vi "PicoScope2000aOpen.vi"(4 "Serial Number":string, 6 "Use Serial Number":bool, 7 "error in (no error)":errorcluster) -> (0 "Max Adc value":i16, 1 "handle":i16, 3 "error out":errorcluster, 5 "Device Info":T1)   [LabVIEW 2010]
doc: "This VI opens a PicoScope 3000a/b and returns a handle to the device."
uses:
  ps2000a.dll
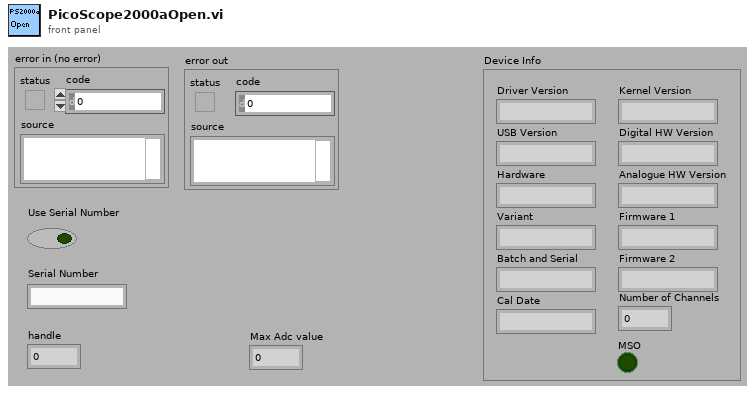
[diagram p1: front panel]
types:
  T1 = cluster{"Driver Version":string, "USB Version":string, "Hardware":string, "Variant":string, "Batch and Serial":string, "Cal Date":string, "Kernel Version":string, "Digital HW Version":string, "Analogue HW Version":string, "Firmware 1":string, "Firmware 2":string, "MSO":bool, "Number of Channels":i16}
  T2 = cluster{"Driver Version":string, "USB Version":string, "Hardware":string, "Variant":string, "Batch and Serial":string, "Cal Date":string, "Kernel Version":string, "Digital HW Version":string, "Analogue HW Version":string, "Firmware 1":string, "Firmware 2":string}
  T3 = cluster{"Driver Version":string, "USB Version":string, "Hardware":string, "Variant":string, "Batch and Serial":string, "Cal Date":string, "Kernel Version":string, "Digital HW Version":string, "Analogue HW Version":string, "Firmware 1":string, "Firmware 2":string, bool, i16}
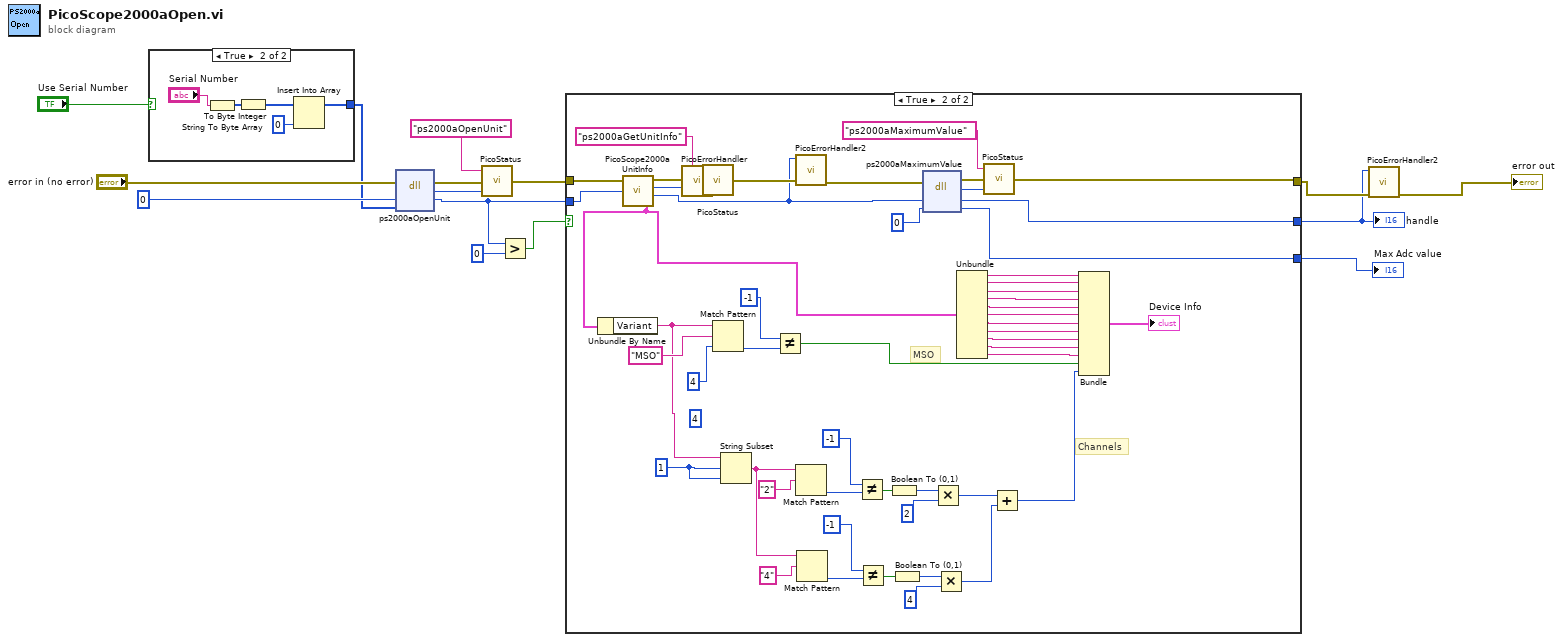
[diagram p0: block diagram]
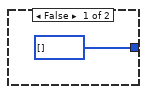
[diagram p2: hidden frame]
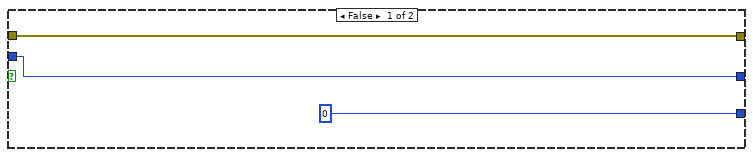
[diagram p3: hidden frame]
diagram:
  n1 = case shown="True" "Use Serial Number" {
    tunnel: [i8[] [] ("serial") w18] -> w1
    frame False {
    }
    frame True {
      n2 = String To Byte Array(string="Serial Number") -> (unsigned byte array=w21:u8[])
      n3 = To Byte Integer(number=w21) -> (8bit integer=w20:i8[])
      n4 = Insert Into Array(array=w20, new element=i8 0 ("new element/subarray")) -> (w18:i8[])  [unwired: 1 in]
    }
  }
  n5 = dll-call lib="ps2000a.dll" fn="ps2000aOpenUnit" ("ps3000.dll:_ps3000_open_unit@0")(error in="error in (no error)", "handle"=i16 0, "serial"=w1) -> (error out=w6:errorcluster, "PICO_STATUS"=w3:u32, "handle"=w2:i16)  [unwired: 3 in, 1 out]
  n6 = call "PicoStatus.vi"("PICO STATUS"=w3, "error in"=w6, "source"="ps2000aOpenUnit") -> ("error out"=w12:errorcluster)
  n7 = Greater?(x=w2, y=i16 0) -> (0:w14:bool)
  n8 = case shown="True" w14 {
    tunnel: w2 -> [w23 w73]
    tunnel: w12 -> [w24 w74]
    tunnel: [w24 w28] -> w10
    tunnel: [w23 w69] -> w8
    tunnel: [i16 0 ("value") w70] -> w11
    frame False {
    }
    frame True {
      w47 = 1 ("offset (0)")
      (unwired) 4 ("offset (0)")
      # "MSO"
      # "Channels"
      n9 = call "PicoScope2000aUnitInfo.vi"("error in (no error)"=w74, "handle in"=w73) -> ("error out"=w72:errorcluster, "PICO_STATUS"=w71:u32, "handle out"=w25:i16, "Unit Info"=w59:T2)  [unwired: 1 in]
      n10 = Unbundle By Name(w59) -> ("Variant"=w31:string)
      n11 = call "PicoStatus.vi"("PICO STATUS"=w71, "error in"=w72, "source"="ps2000aGetUnitInfo") -> ("error out"=w27:errorcluster)
      n12 = Match Pattern(string=w31, regular expression="MSO", offset (0)=4) -> (offset past match=w63:i32)  [unwired: 3 out]
      n13 = String Subset(string=w31, offset (0)=w47, length (rest)=w47) -> (substring=w40:string)
      n14 = Not Equal?(x=-1, y=w63) -> (x != y?=w60:bool)
      n15 = call "PicoErrorHandler2.vi"("error in (no error)"=w27, "handle In"=w25) -> ("error out"=w26:errorcluster)  [unwired: 9 in]
      n16 = Match Pattern(string=w40, regular expression="2") -> (offset past match=w45:i32)  [unwired: 1 in, 3 out]
      n17 = Match Pattern(string=w40, regular expression="4") -> (offset past match=w42:i32)  [unwired: 1 in, 3 out]
      n18 = Not Equal?(x=-1, y=w45) -> (x != y?=w37:bool)
      n19 = Not Equal?(x=-1, y=w42) -> (x != y?=w33:bool)
      n20 = Boolean To (0,1)(Boolean=w37) -> (0, 1=w36:i16)
      n21 = Boolean To (0,1)(Boolean=w33) -> (0, 1=w34:i16)
      n22 = dll-call lib="ps2000a.dll" fn="ps2000aMaximumValue"(error in=w26, "handle"=w25, "value"=i16 0) -> (error out=w67:errorcluster, "PICO_STATUS"=w66:u32, "handle"=w69:i16, "value"=w70:i16)  [unwired: 2 in, 1 out]
      n23 = Multiply(x=w36, y=i16 2) -> (x*y=w39:i16)
      n24 = Multiply(x=w34, y=i16 4) -> (x*y=w32:i16)
      n25 = Unbundle(w59) -> ("Driver Version"=w48:string, "USB Version"=w49:string, "Hardware"=w50:string, "Variant"=w51:string, "Batch and Serial"=w52:string, "Cal Date"=w53:string, "Kernel Version"=w54:string, "Digital HW Version"=w55:string, "Analogue HW Version"=w56:string, "Firmware 1"=w57:string, "Firmware 2"=w58:string)
      n26 = call "PicoStatus.vi"("PICO STATUS"=w66, "error in"=w67, "source"="ps2000aMaximumValue") -> ("error out"=w28:errorcluster)
      n27 = Add(x=w39, y=w32) -> (x+y=w30:i16)
      n28 = Bundle("Driver Version"=w48, "USB Version"=w49, "Hardware"=w50, "Variant"=w51, "Batch and Serial"=w52, "Cal Date"=w53, "Kernel Version"=w54, "Digital HW Version"=w55, "Analogue HW Version"=w56, "Firmware 1"=w57, "Firmware 2"=w58, w60, w30) -> (→"Device Info":T3)  [unwired: 1 in]
    }
  }
  "handle" <- w8
  "Max Adc value" <- w11
  n29 = call "PicoErrorHandler.vi"() -> ()  [unwired: 1 in, 1 out]
  n30 = call "PicoErrorHandler2.vi"("error in (no error)"=w10, "handle In"=w8) -> ("error out"=→"error out":errorcluster)  [unwired: 9 in]
